vi "ZM-CP-UDP-closeConnection.vi"(8 "error in (no error)":errorcluster, 11 "ZM-CP-communication_protocol in":refnum<class "ZM-CP-communication_protocol.lvclass">) -> (0 "error out":errorcluster, 3 "ZM-CP-communication_protocol out":refnum<class "ZM-CP-communication_protocol.lvclass">)   [LabVIEW 2020, in "ZM-CP-UDP-udp_transport.lvlib" / "ZM-CP-UDP-sender.lvclass"]
doc: "Hook of the UDP sender, called by its ZM-CP-close override before Call Parent: closes the UDP connection. The class terminals are typed as the parent so the hook fits the override's class wire."
uses:
  ZM-CP-UDP-sender.lvclass
  ZM-CP-communication_protocol/ZM-CP-communication_protocol/ZM-CP-communication_protocol.lvclass
  ZM-CP-UDP-sender.lvclass/ZM-CP-UDP-sender.ctl
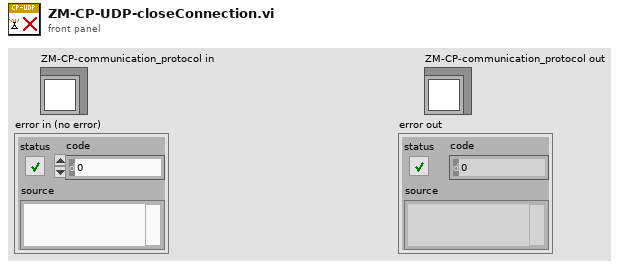
[diagram p1: front panel]
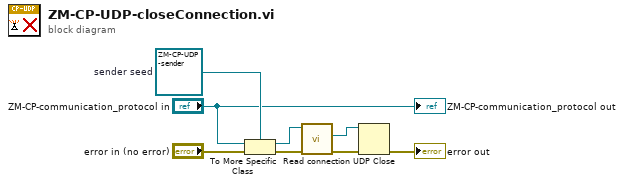
[diagram p0: block diagram]
diagram:
  w7 = refnum<class "ZM-CP-UDP-sender.lvclass"> refnum  # sender seed
  n1 = To More Specific Class(target class=w7, reference="ZM-CP-communication_protocol in", error in="error in (no error)") -> (specific class reference=w5:refnum<class "ZM-CP-UDP-sender.lvclass">, error out=w6:errorcluster)
  n2 = call "Read connection.vi"("error in (no error)"=w6, "ZM-CP-UDP-sender in"=w5) -> ("error out"=w3:errorcluster, "connection"=w4:refnum<k16>)  [unwired: 7 in, 1 out]
  n3 = UDP Close(connection ID=w4, 8:w3) -> (error out=→"error out":errorcluster)  [unwired: 1 out]
  "ZM-CP-communication_protocol out" <- "ZM-CP-communication_protocol in"
